vi "Log.vi"(8 "error in":errorcluster, 10 "Log Entry":T1 {"Time" format="%<%x %.3X>T"}, 11 "UI Logger in":refnum<class "UI Logger.lvclass">) -> (0 "error out":errorcluster, 3 "UI Logger out":refnum<class "UI Logger.lvclass">)   [LabVIEW 2026, in "UI Logger.lvlib" / "UI Logger.lvclass"]
doc: "Log the provided entry."
uses:
  UI Logger.lvclass
  Type Definitions/Log Entry--cluster.ctl
  UI Logger.lvclass/UI Logger.ctl
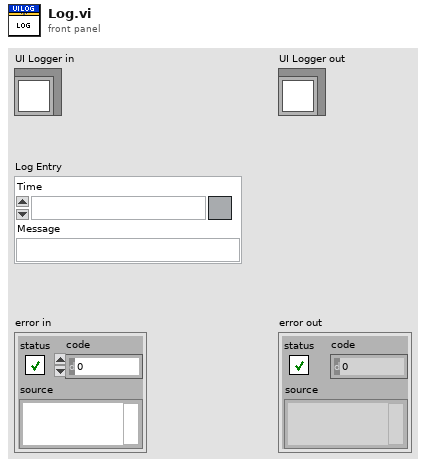
[diagram p1: front panel]
types:
  T1 = typedef "Log Entry--cluster.ctl" = cluster{"Time":timestamp, "Message":string}
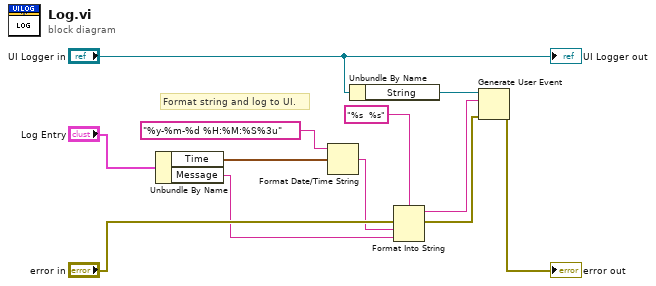
[diagram p0: block diagram]
diagram:
  # "Format string and log to UI."
  n1 = Unbundle By Name("Log Entry") -> ("Time"=w9:timestamp, "Message"=w5:string)
  n2 = Format Date/Time String(time format string (%c)="%y-%m-%d %H:%M:%S%3u", seconds (now)=w9) -> (date/time string=w6:string)  [unwired: 1 in]
  n3 = Unbundle By Name("UI Logger in") -> ("String"=w2:refnum<user-event>)
  n4 = Format Into String(format string="%s  %s", error in="error in", w6, w5) -> (resulting string=w1:string, error out=w11:errorcluster)  [unwired: 1 in]
  n5 = Generate User Event(user event=w2, event data cluster=w1, error in=w11) -> (error out=→"error out":errorcluster)  [unwired: 1 in, 1 out]
  "UI Logger out" <- "UI Logger in"
